vi "FuncVI-FileDelete.vi"(5 "InstanceRef":T2, 9 "arg list":T1[](array[typedef]) {"num" format="%.2f"}) -> (0 "error out":bool, 3 "result":T1 {"num" format="%.2f"})   [LabVIEW 2021]
doc: "::: CalcExpress Toolkit :::\nCopyright (c) 2000-2026 Konstantin Shifershteyn. All rights reserved."
uses:
  cetypes.llb/CalcExpress Function Argument Info.ctl
  cetypes.llb/CalcExpress Instance RefNum.ctl
panel:
  in  "max arg num":i32=1
  in  "min arg num":i32=1
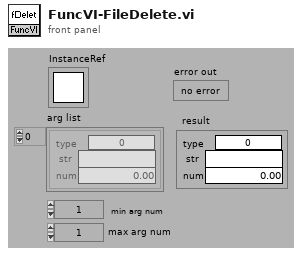
[diagram p1: front panel]
types:
  T1 = typedef "CalcExpress Function Argument Info.ctl" = cluster{"type":u32, "str":string, "num":dbl}
  T2 = typedef "CalcExpress Instance RefNum.ctl" = refnum<k1>
  T3 = enum32{"String", "DBL Number", "identifier", "1D Array of DBL", "2D Array of DBL", "CDB Number", "1D Array of CDB", "2D Array of CDB", "1D Array of String", "2D Array of String", "Unknown data type"}
  T4 = enum32{"existing file", "new file", "new or existing file", "existing dir", "new dir", "new or existing dir", "existing file (use LLBs)", "new file (use LLBs)", "new or existing file (use LLBs)", "new or existing file or directory (use LLBs)", "existing dir (use LLBs)", "new dir (use LLBs)", "new or existing dir (use LLBs)", "existing file or dir", "new file or dir", "new or existing file or dir", "existing file or dir (use LLBs)", "new file or dir (use LLBs)"}
  T5 = cluster{"type: use this constant to specify a predefined type code":enum32{"String", "DBL Number", "identifier", "1D Array of DBL", "2D Array of DBL", "CDB Number", "1D Array of CDB", "2D Array of CDB", "1D Array of String", "2D Array of String", "Unknown data type"}, string, "code":dbl}
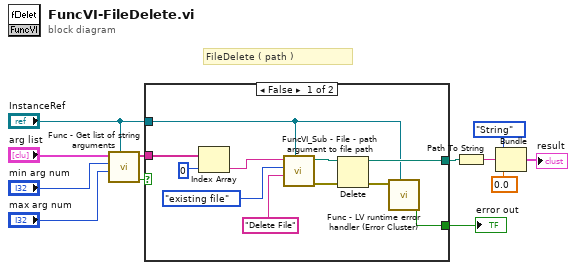
[diagram p0: block diagram]
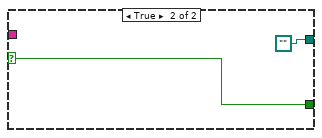
[diagram p2: hidden frame]
diagram:
  # "FileDelete ( path )"
  n1 = call "Func - Get list of string arguments.vi"("InstanceRef"="InstanceRef", "max arg num"="max arg num", "min arg num"="min arg num", "arg list"="arg list") -> ("error out"=w8:bool, "val list"=w9:string[])  [unwired: 4 in]
  n2 = case shown="False" w8 {
    selector: w8 -> [_ w25]
    tunnel: [w13 w25] -> w12
    tunnel: "InstanceRef" -> [w14 _]
    tunnel: w9 -> [w21 _]
    tunnel: [w16 path ""] -> w4
    frame False {
      n3 = Index Array(array=w21, index=0) -> (element=w22:string)
      n4 = call "FuncVI_Sub - File - path argument to file path.vi"("InstanceRef"=w14, "prompt"="Delete File", "select mode (2)"=T4."existing file", "arg: file path"=w22) -> ("error out"=w19:errorcluster, "file path"=w20:path)  [unwired: 5 in, 1 out]
      n5 = Delete(path (use dialog)=w20, error in=w19) -> (deleted path=w16:path, error out=w15:errorcluster)  [unwired: 3 in, 1 out]
      n6 = call "Func - LV runtime error handler (Error Cluster).vi"("InstanceRef"=w14, "LabVIEW error"=w15) -> ("error out"=w13:bool)  [unwired: 4 in, 3 out]
    }
    frame True {
    }
  }
  "error out" <- w12
  n7 = Path To String(path=w4) -> (string=w5:string)
  n8 = Bundle("type: use this constant to specify a predefined type code"=T3."String", w5, "code"=0.0) -> (→"result":T5)  [unwired: 1 in]
